vi "Prepare Checks.vi"(8 "error in":errorcluster, 11 "checks":T2) -> (0 "error out":errorcluster, 3 "Prepared Checks":T1)   [LabVIEW 2026]
doc: "Converts the checks read from a configurable sequence into the form Evaluate All Checks takes. The comparison text becomes the enum. An unknown comparison gives error 5003 so it can never silently act as EQ. AF-free."
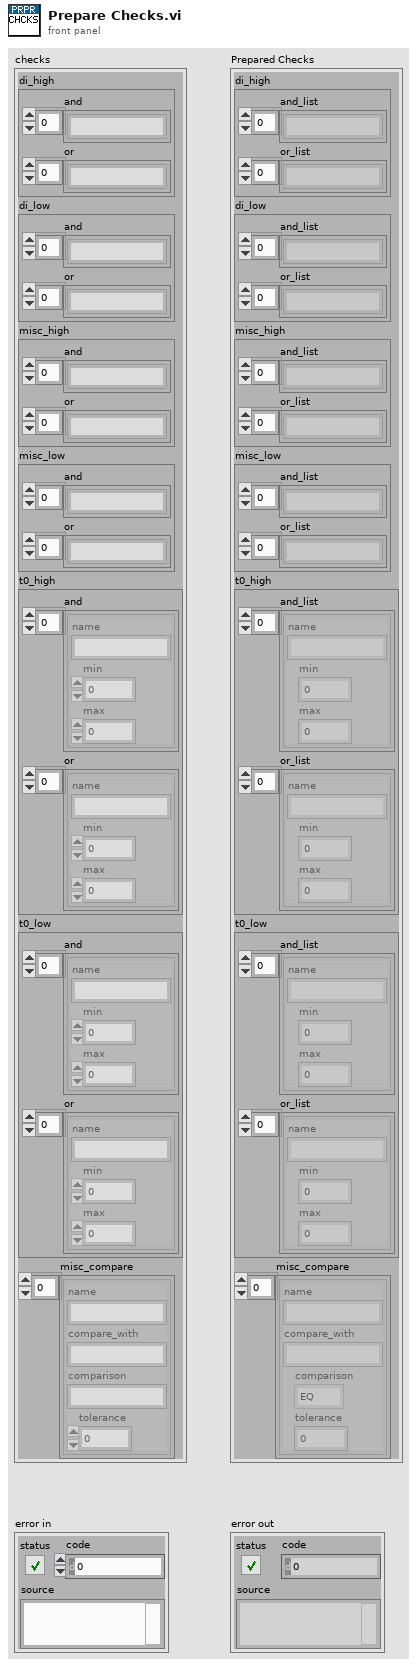
[diagram p1: front panel]
types:
  T1 = cluster{"di_high":cluster{"and_list":string[], "or_list":string[]}, "di_low":cluster{"and_list":string[], "or_list":string[]}, "misc_high":cluster{"and_list":string[], "or_list":string[]}, "misc_low":cluster{"and_list":string[], "or_list":string[]}, "t0_high":cluster{"and_list":cluster{"name":string, "min":dbl, "max":dbl}[], "or_list":cluster{"name":string, "min":dbl, "max":dbl}[]}, "t0_low":cluster{"and_list":cluster{"name":string, "min":dbl, "max":dbl}[], "or_list":cluster{"name":string, "min":dbl, "max":dbl}[]}, "misc_compare":cluster{"name":string, "compare_with":string, "comparison":enum16{"EQ", "NE", "GT", "GE", "LT", "LE"}, "tolerance":dbl}[]}
  T2 = cluster{"di_high":cluster{"and":string[], "or":string[]}, "di_low":cluster{"and":string[], "or":string[]}, "misc_high":cluster{"and":string[], "or":string[]}, "misc_low":cluster{"and":string[], "or":string[]}, "t0_high":cluster{"and":cluster{"name":string, "min":dbl, "max":dbl}[], "or":cluster{"name":string, "min":dbl, "max":dbl}[]}, "t0_low":cluster{"and":cluster{"name":string, "min":dbl, "max":dbl}[], "or":cluster{"name":string, "min":dbl, "max":dbl}[]}, "misc_compare":cluster{"name":string, "compare_with":string, "comparison":string, "tolerance":dbl}[]}
  T3 = cluster{"and":cluster{"name":string, "min":dbl, "max":dbl}[], "or":cluster{"name":string, "min":dbl, "max":dbl}[]}
  T4 = cluster{"name":string, "compare_with":string, "comparison":string, "tolerance":dbl}[]
  T5 = cluster{"name":string, "compare_with":string, "comparison":enum16{"EQ", "NE", "GT", "GE", "LT", "LE"}, "tolerance":dbl}
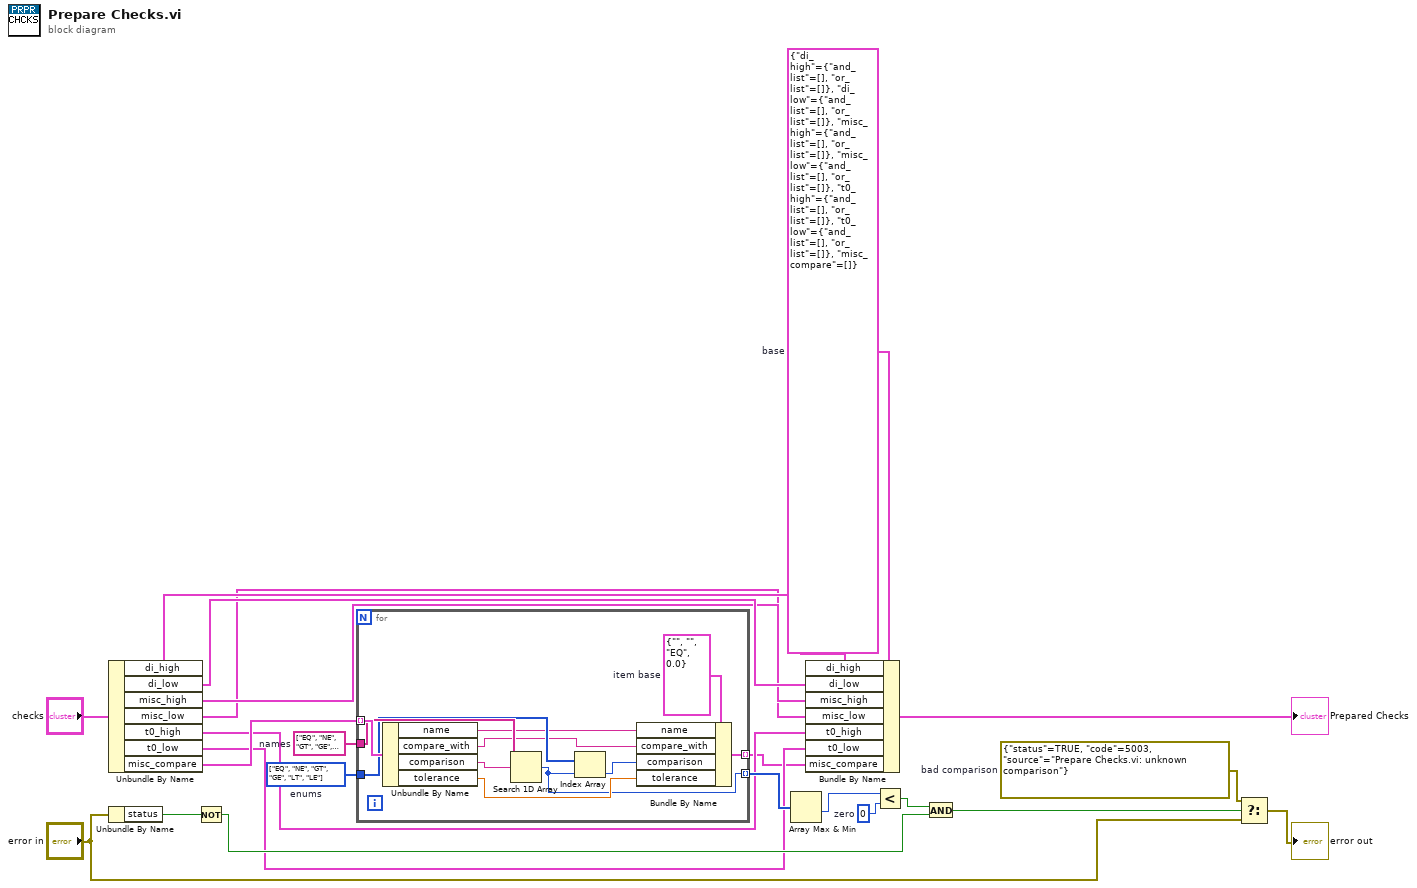
[diagram p0: block diagram]
diagram:
  w17 = 0  # zero
  w13 = errorcluster {"status"=TRUE, "code"=5003, "source"="Prepare Checks.vi: unknown comparison"}  # bad comparison
  w3 = T1 {"di_high"={"and_list"=[], "or_list"=[]}, "di_low"={"and_list"=[], "or_list"=[]}, "misc_high"={"and_list"=[], "or_list"=[]}, "misc_low"={"and_list"=[], "or_list"=[]}, "t0_high"={"and_list"=[], "or_list"=[]}, "t0_low"={"and_list"=[], "or_list"=[]}, "misc_compare"=[]}  # base
  w20 = enum16{"EQ", "NE", "GT", "GE", "LT", "LE"}[] [enum."EQ", enum."NE", enum."GT", enum."GE", enum."LT", enum."LE"] items=["EQ", "NE", "GT", "GE", "LT", "LE"]  # enums
  w21 = string[] ["EQ", "NE", "GT", "GE", "LT", "LE"]  # names
  n1 = Unbundle By Name("checks") -> ("di_high"=w10:cluster{"and":string[], "or":string[]}, "di_low"=w9:cluster{"and":string[], "or":string[]}, "misc_high"=w8:cluster{"and":string[], "or":string[]}, "misc_low"=w7:cluster{"and":string[], "or":string[]}, "t0_high"=w6:T3, "t0_low"=w5:T3, "misc_compare"=w22:T4)
  n2 = Unbundle By Name("error in") -> ("status"=w16:bool)
  n3 = Not(x=w16) -> (.not. x?=w14:bool)
  n4 = for {
    tunnel: w22 -> [w34] mode=indexing
    tunnel: w21 -> [w33]
    tunnel: w20 -> [w31]
    tunnel: [w25] -> w4 mode=indexing
    tunnel: [w24] -> w19 mode=indexing
    w26 = T5 {"name"="", "compare_with"="", "comparison"=enum."EQ", "tolerance"=0.0}  # item base
    n5 = Unbundle By Name(w34) -> ("name"=w30:string, "compare_with"=w29:string, "comparison"=w32:string, "tolerance"=w27:dbl)
    n6 = Search 1D Array(1D array=w33, element=w32) -> (index of element=w24:i32)  [unwired: 1 in]
    n7 = Index Array(array=w31, index=w24) -> (element=w28:enum16{"EQ", "NE", "GT", "GE", "LT", "LE"})
    n8 = Bundle By Name(cluster=w26, "name"=w30, "compare_with"=w29, "comparison"=w28, "tolerance"=w27) -> (w25:T5)
  }
  n9 = Array Max & Min(array=w19) -> (min value=w18:i32)  [unwired: 3 out]
  n10 = Bundle By Name(cluster=w3, "di_high"=w10, "di_low"=w9, "misc_high"=w8, "misc_low"=w7, "t0_high"=w6, "t0_low"=w5, "misc_compare"=w4) -> (→"Prepared Checks":T1)
  n11 = Less?(x=w18, y=w17) -> (x < y?=w15:bool)
  n12 = And(x=w15, y=w14) -> (x .and. y?=w12:bool)
  n13 = Select(t=w13, s=w12, f="error in") -> (s? t:f=→"error out":errorcluster)
